vi "Test Helper - Open and Close Client.vi"(8 "error in (no error)":errorcluster) -> (0 "error out":errorcluster)   [LabVIEW 2019, in "RemoteControl.ZMQ.Tests.lvclass"]
uses:
  RemoteControl.ZMQ.Tests.lvclass
  C:/Program Files/National Instruments/LabVIEW 2019/user.lib/LevyLab/RemoteControl/RemoteControl/RemoteControl.lvclass
  <userlib>/LevyLab/RemoteControl/RemoteControl/RemoteControl.lvclass
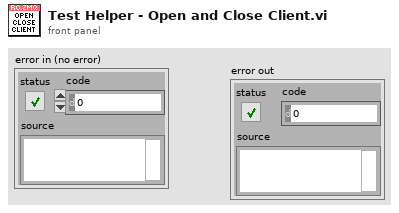
[diagram p1: front panel]
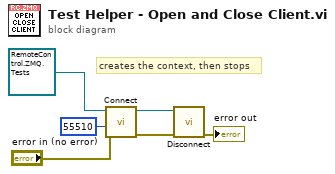
[diagram p0: block diagram]
diagram:
  # "creates the context, then stops"
  n1 = call <userlib>:"Connect.vi"("error in (no error)"="error in (no error)", "Port"=u16 55510, "RemoteControl in"=refnum<class "RemoteControl.ZMQ.Tests.lvclass"> refnum ("RemoteControl.ZMQ.Tests.lvclass")) -> ("error out"=w1:errorcluster, "RemoteControl out"=w5:refnum<class "RemoteControl.ZMQ.Tests.lvclass">)  [unwired: 7 in]
  n2 = call <userlib>:"Disconnect.vi"("error in (no error)"=w1, "RemoteControl in"=w5) -> ("error out"=→"error out":errorcluster)  [unwired: 8 in, 1 out]
